vi "Write connection.vi"(8 "error in (no error)":errorcluster, 10 "connection":refnum<k16>, 11 "ZM-CP-UDP-receiver in":refnum<class "ZM-CP-UDP-receiver.lvclass">) -> (0 "error out":errorcluster, 3 "ZM-CP-UDP-receiver out":refnum<class "ZM-CP-UDP-receiver.lvclass">)   [LabVIEW 2020, in "ZM-CP-UDP-udp_transport.lvlib" / "ZM-CP-UDP-receiver.lvclass"]
doc: "Writes one field of this class's private data. Generated by lvai_create_accessors from the class private data control."
uses:
  ZM-CP-UDP-receiver.lvclass
  ZM-CP-UDP-receiver.lvclass/ZM-CP-UDP-receiver.ctl
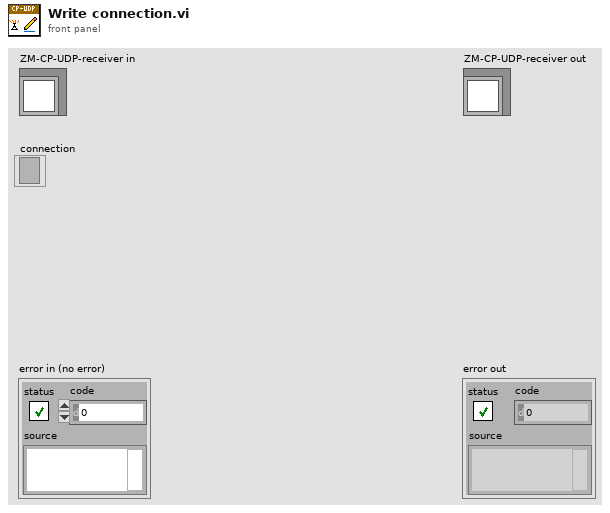
[diagram p1: front panel]
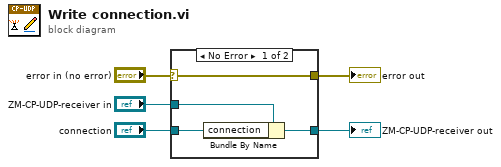
[diagram p0: block diagram]
diagram:
  n1 = case shown="No Error" "error in (no error)" {
    selector: "error in (no error)" -> [w9 w10]
    tunnel: [w9 w10] -> w4
    tunnel: [w7 w11] -> w2
    tunnel: "ZM-CP-UDP-receiver in" -> [w8 w11]
    tunnel: "connection" -> [w6 _]
    frame No Error {
      n2 = Bundle By Name(cluster=w8, "connection"=w6) -> (w7:refnum<class "ZM-CP-UDP-receiver.lvclass">)
    }
    frame Error {
    }
  }
  "error out" <- w4
  "ZM-CP-UDP-receiver out" <- w2
